vi "Frame_Draw.vi"(0 "State":T4={"Tick"=0, "Phase"=0, "PhaseTicks"=0, "Level"=1, "Room"=0, "X10"=0, "Y10"=0, "VY10"=0, "Mode"=0, "Facing"=0, "Run"=0, "Vert"=0, "StandY"=0, "EntryX10"=0, "EntryY10"=0, "EntryMode"=0, "Lives"=4, "Score"=0, "NextLife"=10000, "KeyR"=0, "KeyB"=0, "KeyY"=0, "Torch"=FALSE, "FloorPhase"=0, "Dead"=FALSE, "LevelStart"=FALSE, "Quit"=FALSE, "Sound"=0, "Seed"=12345, "DemoStep"=0, "Tiles"=[], "World"=[], "Enemies"=[], "Highscores"=[], "Name"=[0, 0, 0], "Cursor"=0}, 1 "Memory":T1={"RoomKey"=-1, "Key"=-1, "NameKey"=-1, "Lit"=[], "Dim"=[], "Dark"=[], "Comp"=[], "Template"={"image type"=0, "image depth"=0, "image"=[], "mask"=[], "colors"=[], "Rectangle"={"left"=0, "top"=0, "right"=0, "bottom"=0}}, "CX"=-1, "CY"=-1, "X1"=0, "Y1"=0, "X2"=0, "Y2"=0, "Prev"=[], "HudKey"=-1, "HudScore"=-1, "HudTime"=-1, "Full"=[]}, 5 "Sprites":cluster{"Pix":u8[][], "Mask":u8[][]}[](array[cluster]), 7 "Hud":T3, 9 "Title":T3, 11 "error in":errorcluster) -> (4 "Picture":picture, 6 "Pieces":T2(array[cluster]), 8 "Memory out":T1={"RoomKey"=-1, "Key"=-1, "NameKey"=-1, "Lit"=[], "Dim"=[], "Dark"=[], "Comp"=[], "Template"={"image type"=0, "image depth"=0, "image"=[], "mask"=[], "colors"=[], "Rectangle"={"left"=0, "top"=0, "right"=0, "bottom"=0}}, "CX"=-1, "CY"=-1, "X1"=0, "Y1"=0, "X2"=0, "Y2"=0, "Prev"=[], "HudKey"=-1, "HudScore"=-1, "HudTime"=-1, "Full"=[]}, 15 "error out":errorcluster)   [LabVIEW 2020, in "GH_Render.lvlib"]
doc: "Draws one frame: the WHOLE screen every frame (like Pauls Hoehenflug) - every update of the picture control is complete, so nothing can stay behind and LabVIEW may skip frames without harm. Room_Grid gives the room raster (Memory keeps the room pictures and the composite of a dark room), Claude_View what is drawn of Claude, Scene_Blit builds the screen raster, one Draw Flattened Pixmap shows it. Pieces stays empty (kept for the interface)."
uses:
  GH_Render.lvlib
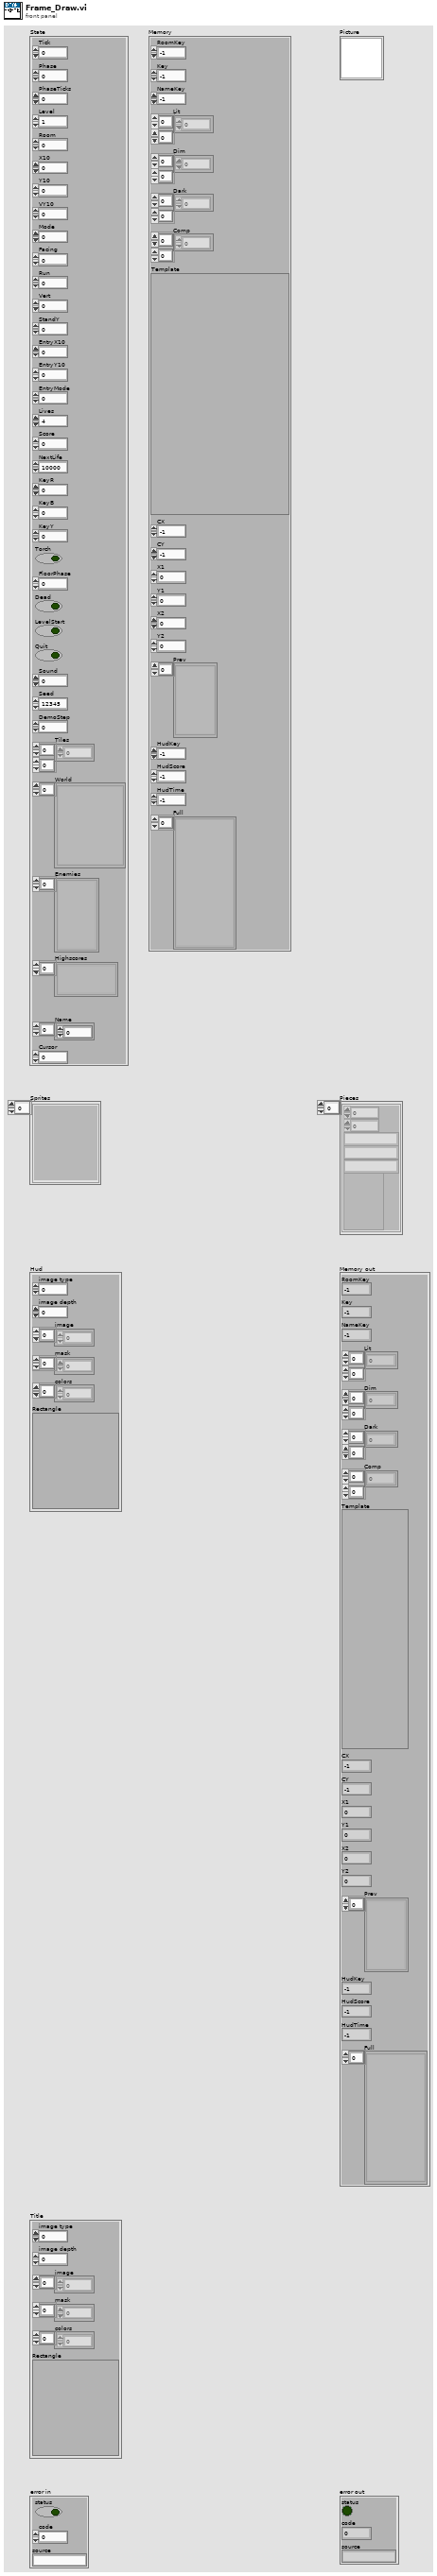
[diagram p1: front panel]
types:
  T1 = cluster{"RoomKey":i32, "Key":i32, "NameKey":i32, "Lit":u8[][], "Dim":u8[][], "Dark":u8[][], "Comp":u8[][], "Template":cluster{"image type":i32, "image depth":i32, "image":u8[], "mask":u8[], "colors":u32[], "Rectangle":cluster{"left":i16, "top":i16, "right":i16, "bottom":i16}}, "CX":i32, "CY":i32, "X1":i32, "Y1":i32, "X2":i32, "Y2":i32, "Prev":cluster{"Kind":i32, "X10":i32, "Y10":i32, "Dir":i32, "Mode":i32}[], "HudKey":i32, "HudScore":i32, "HudTime":i32, "Full":cluster{"image type":i32, "image depth":i32, "image":u8[], "mask":u8[], "colors":u32[], "Rectangle":cluster{"left":i16, "top":i16, "right":i16, "bottom":i16}}[]}
  T2 = cluster{"image type":i32, "image depth":i32, "image":u8[], "mask":u8[], "colors":u32[], "Rectangle":cluster{"left":i16, "top":i16, "right":i16, "bottom":i16}}[]
  T3 = cluster{"image type":i32, "image depth":i32, "image":u8[], "mask":u8[], "colors":u32[], "Rectangle":cluster{"left":i16, "top":i16, "right":i16, "bottom":i16}}
  T4 = cluster{"Tick":u32, "Phase":i32, "PhaseTicks":i32, "Level":i32, "Room":i32, "X10":i32, "Y10":i32, "VY10":i32, "Mode":i32, "Facing":i32, "Run":i32, "Vert":i32, "StandY":i32, "EntryX10":i32, "EntryY10":i32, "EntryMode":i32, "Lives":i32, "Score":i32, "NextLife":i32, "KeyR":i32, "KeyB":i32, "KeyY":i32, "Torch":bool, "FloorPhase":i32, "Dead":bool, "LevelStart":bool, "Quit":bool, "Sound":i32, "Seed":u32, "DemoStep":i32, "Tiles":u8[][], "World":cluster{"ID":string, "Depth":i32, "Column":i32, "Tiles":u8[][]}[], "Enemies":cluster{"Kind":i32, "X10":i32, "Y10":i32, "Dir":i32, "Mode":i32}[], "Highscores":cluster{"Score":i32, "Name":string}[], "Name":i32[], "Cursor":i32}
  T5 = cluster{"left":i16, "top":i16, "right":i16, "bottom":i16}
  T6 = cluster{"Hide":bool, "CX":i32, "CY":i32, "ClaudeIdx":i32, "ClaudeX":i32, "ClaudeY":i32}
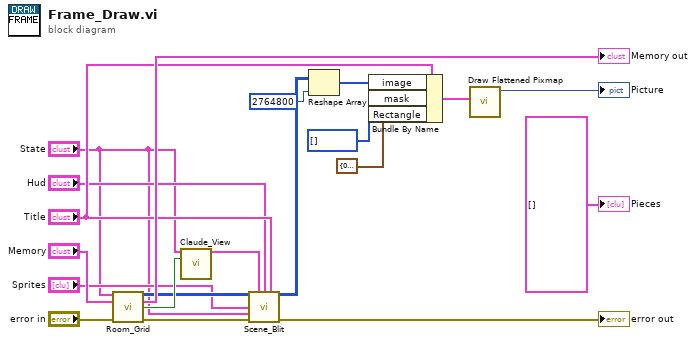
[diagram p0: block diagram]
diagram:
  n1 = call "Room_Grid.vi"("State"="State", "Memory"="Memory", "error in"="error in") -> ("Grid"=w7:u8[][], "Memory out"=→"Memory out":T1, "Dark"=w9:bool, "error out"=w10:errorcluster)  [unwired: 9 in]
  n2 = call "Claude_View.vi"("State"="State", "Dark"=w9) -> ("View"=w11:T6)  [unwired: 13 in]
  n3 = call "Scene_Blit.vi"("Grid"=w7, "View"=w11, "Hud"="Hud", "Title"="Title", "Sprites"="Sprites", "State"="State", "error in"=w10) -> ("Picture"=w12:u8[][], "error out"=→"error out":errorcluster)  [unwired: 7 in]
  n4 = Reshape Array(w12, 2764800) -> (w15:u8[])
  n5 = Bundle By Name(cluster="Title", "image"=w15, "mask"=u8[] [], "Rectangle"=T5 {"left"=0, "top"=0, "right"=1280, "bottom"=720}) -> (w18:T3)
  n6 = call <vilib>:"Draw Flattened Pixmap.vi"("image data"=w18) -> ("new picture"=→"Picture":picture)  [unwired: 8 in]
  "Pieces" <- T2 [] ("No pieces")
